vi "Document Property Node.vi"   [LabVIEW 2017]
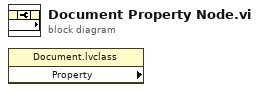
[diagram p0: block diagram]
diagram:
  n1 = property class="Document.lvclass" props=[]() -> ()  [unwired: 2 in, 3 out]
